vi "GetItemInfo.vi"(11 "Num MRU Items":u16=10) -> (0 "Mode XML Elements":string, 1 "ring info":refnum<class "RingItem.lvclass">[](array[class]), 3 "item info array":T1(array[cluster]))   [LabVIEW 2023, in "GettingStartedWindow.lvlib"]
uses:
  <resource>/modes/FRC/GSW/GettingStartedWindow.lvlib
  <resource>/modes/FRC/GSW/Classes/ClickableText/ClickableText.lvclass
  home/systemcore/natinst/lvaddons/wpilib/1/resource/modes/FRC/GSW/Classes/Link/Link.lvclass
  <resource>/modes/FRC/GSW/Classes/RingItem/RingItem.lvclass
  <resource>/modes/FRC/GSW/Classes/MRU/MRU.lvclass
  home/systemcore/natinst/lvaddons/wpilib/1/resource/modes/FRC/GSW/Classes/ClickableText/ClickableText.lvclass
  <resource>/modes/FRC/GSW/Classes/Separator/Separator.lvclass
  <resource>/modes/FRC/GSW/Classes/Link/Link.lvclass
panel:
  out "Debugging display - ring items - enable code on diagram to view":string[](array[string])
  out "Debugging display - enable code on diagram to view":cluster{string[]}[][](array[cluster])
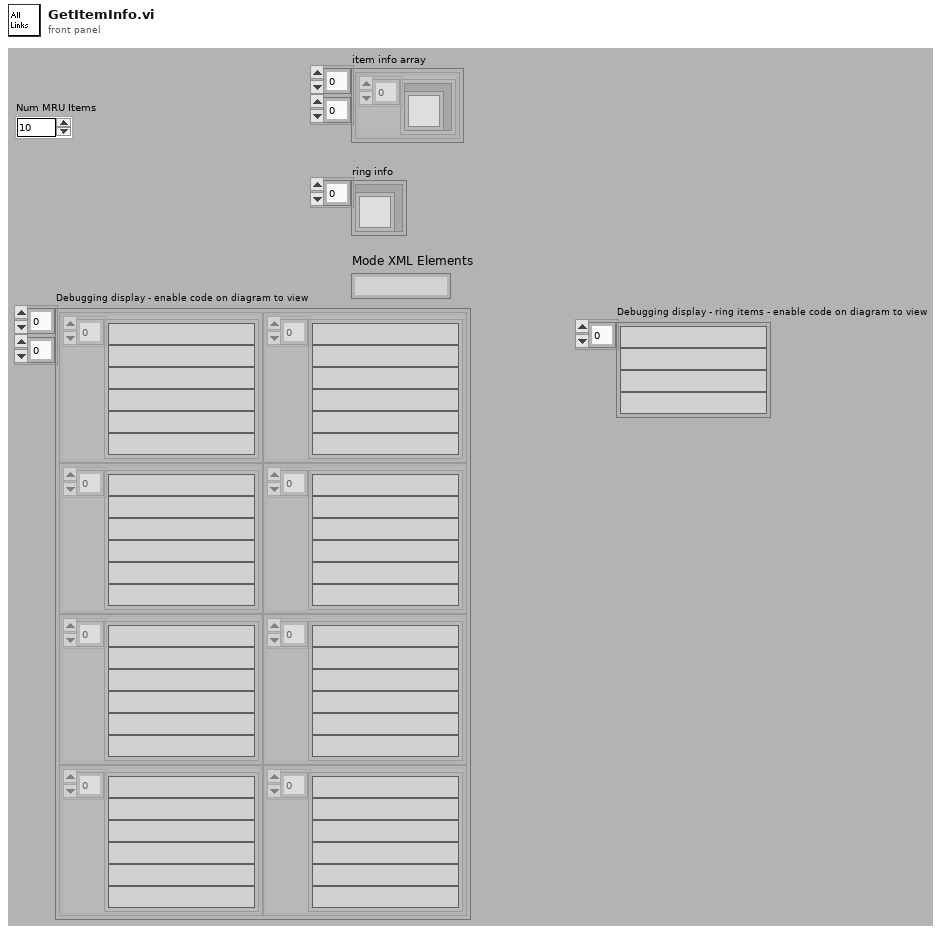
[diagram p1: front panel]
types:
  T1 = cluster{refnum<class "ClickableText.lvclass">[]}[][]
  T2 = typedef "GettingStartedWindow.lvlib/ItemData_Type.ctl" = enum16{"None", "Folder", "New Project", "New VI", "Find", "VI", "Project", "New from template", "RT Project Wizard", "PDA Project Wizard", "Control", "Library", "Class", "XControl", "Runtime menu", "Statechart", "Ladder", "Find LabVIEW Addons", "Instrument Finder", "Example Finder"}
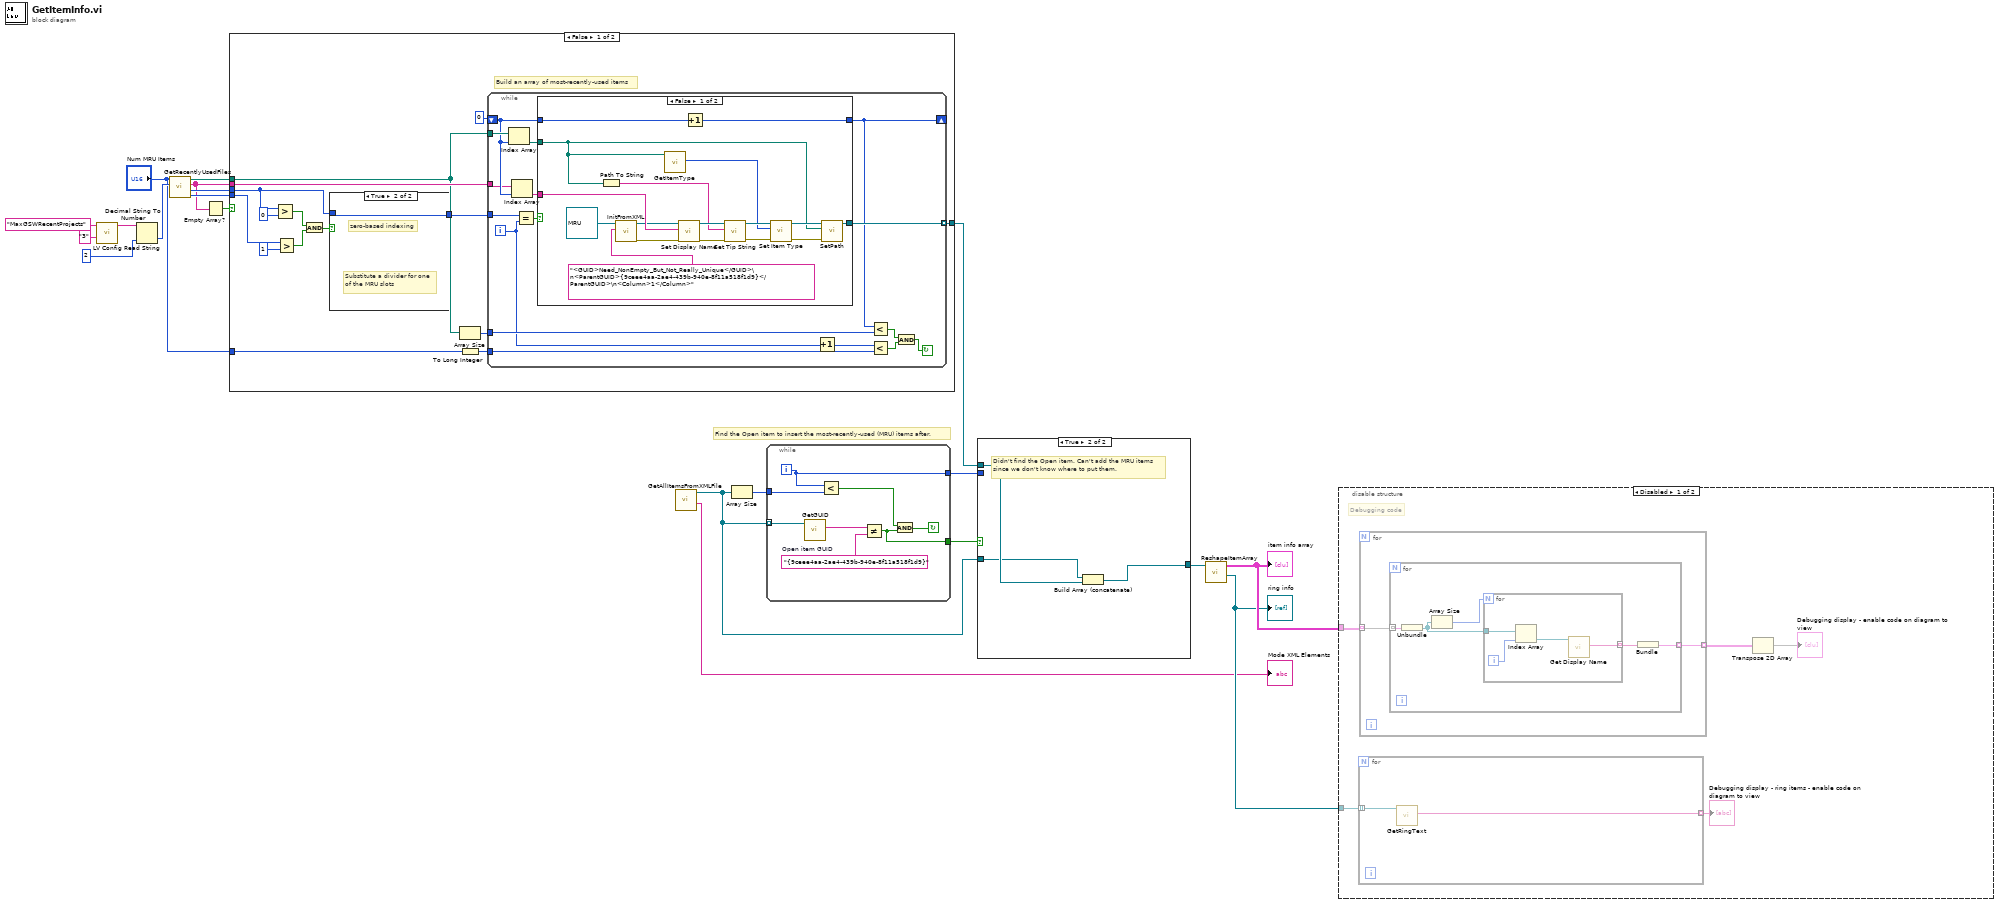
[diagram p0: block diagram]
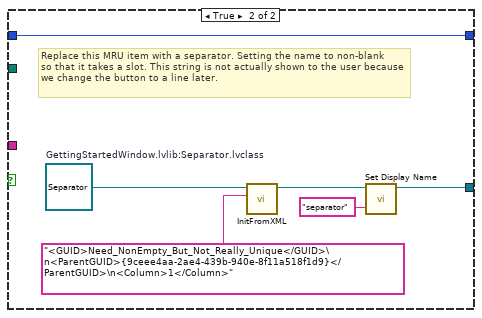
[diagram p2: hidden frame]
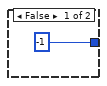
[diagram p3: hidden frame]
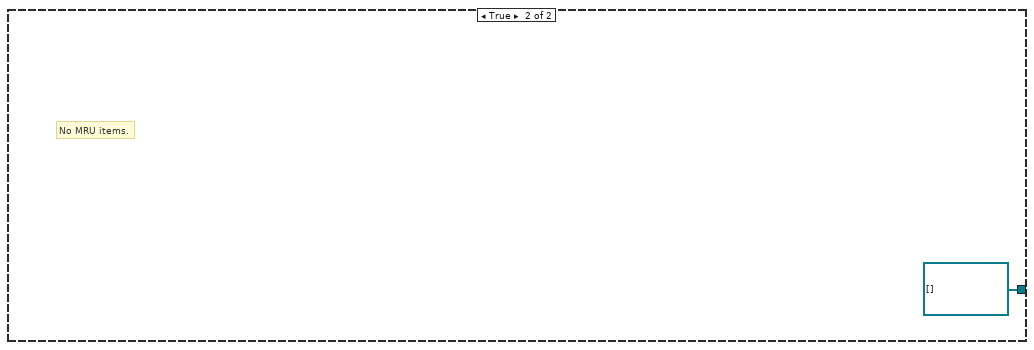
[diagram p4: hidden frame]
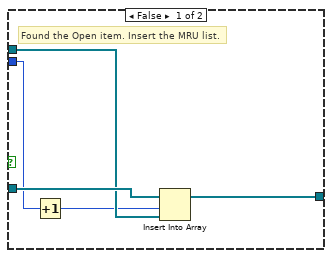
[diagram p5: hidden frame]
diagram:
  # "Find the Open item to insert the most-recently-used (MRU) items after."
  n1 = call <resource>:"LV Config Read String.vi"("default value"="3", "key"="MaxGSWRecentProjects") -> ("value"=w10:string)  [unwired: 2 in, 3 out]
  n2 = Decimal String To Number(string=w10, default (0L)=2) -> (number=w8:i32)  [unwired: 2 out]
  n3 = call <resource>:"GetRecentlyUsedFiles.vi"("Max number of slots for projects (2)"=w8, "Number of available slots"="Num MRU Items") -> ("number of bottom slots"=w7:i32, "number of top slots"=w6:i32, "Recent item names"=w3:string[], "recently used item paths"=w5:path[])  [unwired: 6 out]
  n4 = Empty Array?(array=w3) -> (empty?=w2:bool)
  n5 = case shown="False" w2 {
    tunnel: w3 -> [w35 _]
    tunnel: [w34 refnum<class "ClickableText.lvclass">[] []] -> w18
    tunnel: w7 -> [w32 _]
    tunnel: w6 -> [w27 _]
    tunnel: w5 -> [w24 _]
    tunnel: "Num MRU Items" -> [w22 _]
    frame False {
      # "Build an array of most-recently-used items"
      n6 = Greater?(x=w27, y=0) -> (0:w30:bool)
      n7 = Greater?(x=w32, y=1) -> (0:w29:bool)
      n8 = And(x=w30, y=w29) -> (x .and. y?=w28:bool)
      n9 = case shown="True" w28 {
        tunnel: w27 -> [_ w76]
        tunnel: [-1 w76] -> w26
        frame False {
        }
        frame True {
          # "zero-based indexing"
          # "Substitute a divider for one\nof the MRU slots"
        }
      }
      n10 = Array Size(array=w24) -> (size(s)=w23:i32)
      n11 = To Long Integer(number=w22) -> (32bit integer=w21:i32)
      n12 = while {
        tunnel: w35 -> [w44]
        tunnel: w24 -> [w51]
        tunnel: [w50] -> w34 mode=indexing
        tunnel: w26 -> [w49]
        shift-right: [w40] -> _
        shift-left: 0 -> [w45]
        tunnel: w23 -> [w43]
        tunnel: w21 -> [w39]
        i -> [w37]
        stop <- w41 continue-if-true
        n13 = Index Array(array=w51, index=w45) -> (element=w47:path)
        n14 = Index Array(array=w44, index=w45) -> (element=w46:string)
        n15 = Equal?(x=w49, y=w37) -> (x = y?=w48:bool)
        n16 = case shown="False" w48 {
          tunnel: w46 -> [w68 _]
          tunnel: w47 -> [w59 _]
          tunnel: [w54 w74] -> w50
          tunnel: w45 -> [w53 w69]
          tunnel: [w52 w69] -> w40
          frame False {
            n17 = Path To String(path=w59) -> (string=w66:string)
            n18 = call-dynamic "InitFromXML.vi"("XML"="<GUID>Need_NonEmpty_But_Not_Really_Unique</GUID>\n<ParentGUID>{9ceee4aa-2ae4-439b-940e-8f11a518f1d9}</ParentGUID>\n<Column>1</Column>", "ClickableText in"=refnum<class "MRU.lvclass"> refnum ("GettingStartedWindow.lvlib:MRU.lvclass")) -> ("error out"=w56:errorcluster, "ClickableText out"=w57:refnum<class "MRU.lvclass">)  [unwired: 1 in, 7 out]
            n19 = call <resource>:"GetItemType.vi"("Path"=w59) -> ("DNL_Type"=w63:T2)  [unwired: 10 out]
            n20 = call <resource>:"Set Display Name.vi"("error in (no error)"=w56, "localized name"=w68, "ClickableText in"=w57) -> ("error out"=w65:errorcluster, "ClickableText out"=w67:refnum<class "MRU.lvclass">)  [unwired: 7 out]
            n21 = Increment(x=w53) -> (x+1=w52:i32)
            n22 = call <resource>:"Set Tip String.vi"("error in (no error)"=w65, "tip string"=w66, "ClickableText in"=w67) -> ("error out"=w62:errorcluster, "ClickableText out"=w64:refnum<class "MRU.lvclass">)  [unwired: 7 out]
            n23 = call <resource>:"Set Item Type.vi"("error in (no error)"=w62, "DNL_Type"=w63, "ClickableText in"=w64) -> ("error out"=w60:errorcluster, "ClickableText out"=w61:refnum<class "MRU.lvclass">)  [unwired: 7 out]
            n24 = call <resource>:"SetPath.vi"("error in (no error)"=w60, "path to MRU item"=w59, "MRU in"=w61) -> ("MRU out"=w54:refnum<class "MRU.lvclass">)  [unwired: 8 out]
          }
          frame True {
            w72 = refnum<class "Separator.lvclass"> refnum  # GettingStartedWindow.lvlib:Separator.lvclass
            # "Replace this MRU item with a separator. Setting the name to non-blank \nso that it takes a slot. This string is not actually shown to the user because \nwe change the button to a line later."
            n25 = call-dynamic "InitFromXML.vi"("XML"="<GUID>Need_NonEmpty_But_Not_Really_Unique</GUID>\n<ParentGUID>{9ceee4aa-2ae4-439b-940e-8f11a518f1d9}</ParentGUID>\n<Column>1</Column>", "ClickableText in"=w72) -> ("ClickableText out"=w71:refnum<class "Separator.lvclass">)  [unwired: 1 in, 8 out]
            n26 = call <resource>:"Set Display Name.vi"("localized name"="separator", "ClickableText in"=w71) -> ("ClickableText out"=w74:refnum<class "Separator.lvclass">)  [unwired: 1 in, 8 out]
          }
        }
        n27 = Increment(x=w37) -> (x+1=w36:i32)
        n28 = Less?(x=w40, y=w43) -> (x < y?=w42:bool)
        n29 = Less?(x=w36, y=w39) -> (x < y?=w38:bool)
        n30 = And(x=w42, y=w38) -> (x .and. y?=w41:bool)
      }
    }
    frame True {
      # "No MRU items."
    }
  }
  n31 = call <resource>:"GetAllItemsFromXMLFile.vi"() -> ("Mode XML Elements"=→"Mode XML Elements":string, "Array"=w16:refnum<class "Link.lvclass">[])  [unwired: 10 out]
  n32 = Array Size(array=w16) -> (size(s)=w20:i32)
  n33 = while {
    tunnel: w20 -> [w80]
    tunnel: w16 -> [w85] mode=indexing
    tunnel: [w79] -> w17
    tunnel: [w78] -> w19
    i -> [w79]
    stop <- w81 continue-if-true
    w83 = "{9ceee4aa-2ae4-439b-940e-8f11a518f1d9}"  # Open item GUID
    n34 = call <resource>:"GetGUID.vi"("Link in"=w85) -> ("GUID"=w84:string)  [unwired: 1 in, 9 out]
    n35 = Less?(x=w79, y=w80) -> (x < y?=w82:bool)
    n36 = Not Equal?(x=w84, y=w83) -> (x != y?=w78:bool)
    n37 = And(x=w82, y=w78) -> (x .and. y?=w81:bool)
  }
  n38 = case shown="True" w19 {
    tunnel: w18 -> [w89 w93]
    tunnel: w17 -> [w88 _]
    tunnel: w16 -> [w90 w91]
    tunnel: [w87 w92] -> w15
    frame False {
      # "Found the Open item. Insert the MRU list."
      n39 = Increment(x=w88) -> (x+1=w86:i32)
      n40 = Insert Into Array(array=w90, index=w86, new element=w89) -> (w87:refnum<class "Link.lvclass">[])
    }
    frame True {
      # "Didn't find the Open item. Can't add the MRU items\nsince we don't know where to put them."
      n41 = Build Array (concatenate)(w91, w93) -> (w92:refnum<class "Link.lvclass">[])
    }
  }
  n42 = call <resource>:"ReshapeItemArray.vi"("Array"=w15) -> ("ring info"=w13:refnum<class "RingItem.lvclass">[], "item info array"=w14:T1)  [unwired: 9 out]
  "item info array" <- w14
  "ring info" <- w13
  n43 = disable-structure shown="Disabled" {
    disable-tunnel: w14 -> [w98 _]
    disable-tunnel: w13 -> [w97 _]
    frame Disabled {
      # "Debugging code"
      n44 = for {
        tunnel: w97 -> [w100] mode=indexing
        tunnel: [w99] -> w96 mode=indexing
        n45 = call <resource>:"GetRingText.vi"("RingItem in"=w100) -> ("ring text"=w99:string)  [unwired: 1 in, 9 out]
      }
      "Debugging display - ring items - enable code on diagram to view" <- w96
      n46 = for {
        tunnel: w98 -> [w102] mode=indexing
        tunnel: [w101] -> w95 mode=indexing
        n47 = for {
          tunnel: w102 -> [w107] mode=indexing
          tunnel: [w103] -> w101 mode=indexing
          n48 = Unbundle(w107) -> (w105:refnum<class "ClickableText.lvclass">[])
          n49 = Array Size(array=w105) -> (size(s)=w106:i32)
          n50 = for {
            N: w106 -> [_]
            tunnel: w105 -> [w111]
            tunnel: [w108] -> w104 mode=indexing
            i -> [w110]
            n51 = Index Array(array=w111, index=w110) -> (element=w109:refnum<class "ClickableText.lvclass">)
            n52 = call-dynamic "Get Display Name.vi"("ClickableText in"=w109) -> ("localized name"=w108:string)  [unwired: 1 in, 9 out]
          }
          n53 = Bundle(w104) -> (w103:cluster{string[]})  [unwired: 1 in]
        }
      }
      n54 = Transpose 2D Array(2D array=w95) -> (transposed array=→"Debugging display - enable code on diagram to view":cluster{string[]}[][])
    }
    frame Enabled {
    }
  }
